vi "MonitorTemperaturaDS18B20.vi"() -> ()   [LabVIEW 2025]
panel:
  in  "stop":bool
  out "Waveform Chart":dbl(graph)
  out "Temperatura °C":dbl
  in  "Puerto":u16=5000
  in  "Dirección IP":string="192.168.4.1"
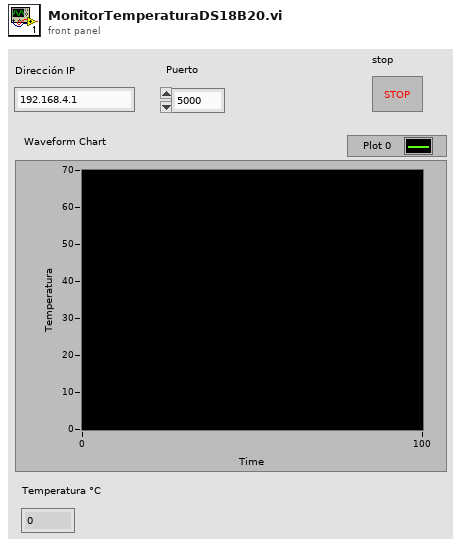
[diagram p1: front panel]
types:
  T1 = enum16{"Standard", "Buffered", "CRLF", "Immediate"}
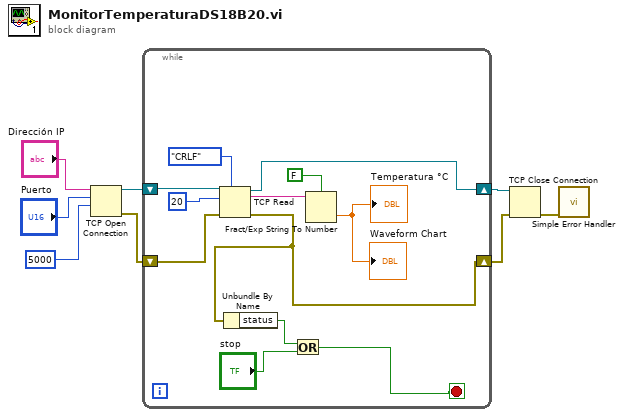
[diagram p0: block diagram]
diagram:
  n1 = TCP Open Connection(address="Dirección IP", remote port or service name="Puerto", timeout ms (60000)=5000) -> (connection ID=w8:refnum<k5>, error out=w7:errorcluster)  [unwired: 2 in]
  n2 = while {
    shift-right: [w15] -> w6
    shift-left: w7 -> [w17]
    shift-right: [w16] -> w5
    shift-left: w8 -> [w20]
    stop <- w9 stop-if-true
    n3 = TCP Read(connection ID=w20, bytes to read=20, error in (no error)=w17, 7:T1."CRLF" ("mode (standard)")) -> (connection ID out=w16:refnum<k5>, data out=w18:string, error out=w15:errorcluster)  [unwired: 1 in]
    n4 = Unbundle By Name(w15) -> ("status"=w14:bool)
    n5 = Or(x=w14, y="stop") -> (x .or. y?=w9:bool)
    n6 = Fract/Exp String To Number(use system decimal point (T)=FALSE, string=w18) -> (number=→"Temperatura °C" →"Waveform Chart":dbl)  [unwired: 2 in, 1 out]
  }
  n7 = TCP Close Connection(connection ID=w5, error in (no error)=w6) -> (error out=w1:errorcluster)  [unwired: 1 in, 1 out]
  n8 = call <vilib>:"Simple Error Handler.vi"("error in (no error)"=w1) -> ()  [unwired: 4 in, 5 out]
